vi "lab2_2.vi"() -> ()   [LabVIEW 2026]
uses:
  <vilib>/rvi/Emulation/niFpgaGetClockAttributes.vi
  <vilib>/rvi/Emulation/niFpgaSctlEmulationGetInTimedLoop.vi
  <vilib>/rvi/Emulation/niFpgaEmulationReportErrorSimple.vi
  <vilib>/rvi/eio/common/nirviEmuTemplateMethod_errors.vi
  <vilib>/rvi/Emulation/niFpgaCriticalErrorInLSC.vi
  <vilib>/eio/EIONode/EIONode.xnode
panel:
  out "AccelerationZ Max":i16
  out "AccelerationY Max":i16
  out "AccelerationX Max":i16
  out "AccelerationZ Now":i16
  out "AccelerationY Now":i16
  out "AccelerationX Now":i16
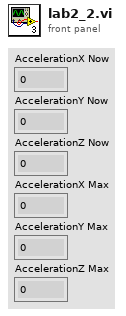
[diagram p1: front panel]
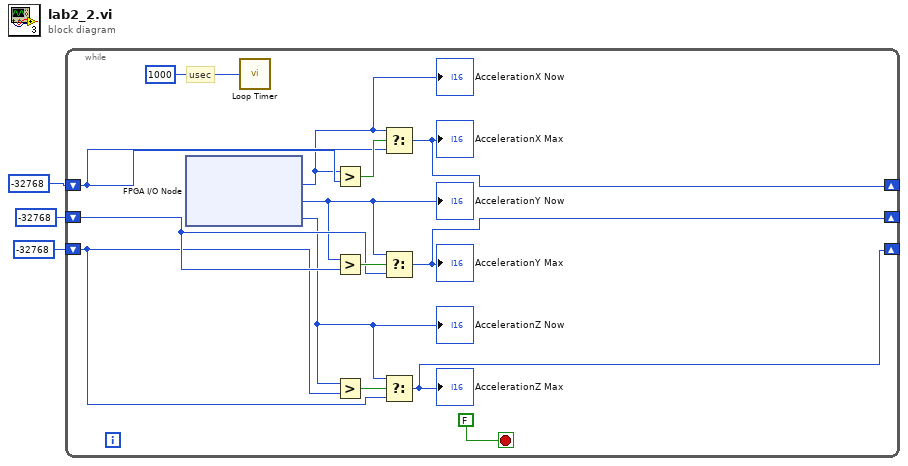
[diagram p0: block diagram]
diagram:
  n1 = while {
    shift-right: [w4] -> _
    shift-left: i16 -32768 ("x") -> [w10]
    shift-right: [w6] -> _
    shift-left: i16 -32768 ("x") -> [w12]
    shift-right: [w5] -> _
    shift-left: i16 -32768 ("x") -> [w11]
    stop <- FALSE stop-if-true
    # "usec"
    n2 = xnode "FPGA I/O Node"() -> ("AccelerationX"=w9:i16, "AccelerationY"=w8:i16, "AccelerationZ"=w7:i16)  [unwired: 3 in, 3 out]
    "AccelerationX Now" <- w9
    "AccelerationY Now" <- w8
    "AccelerationZ Now" <- w7
    n3 = call "Loop Timer"("Count(uSec)"=u32 1000) -> ()  [unwired: 1 out]
    n4 = Greater?(x=w9, y=w12) -> (0:w15:bool)
    n5 = Greater?(x=w8, y=w11) -> (0:w14:bool)
    n6 = Greater?(x=w7, y=w10) -> (0:w13:bool)
    n7 = Select(t=w9, s=w15, f=w12) -> (s? t:f=w6:i16)
    "AccelerationX Max" <- w6
    n8 = Select(t=w8, s=w14, f=w11) -> (s? t:f=w5:i16)
    "AccelerationY Max" <- w5
    n9 = Select(t=w7, s=w13, f=w10) -> (s? t:f=w4:i16)
    "AccelerationZ Max" <- w4
  }
